vi "Update Measurement Details.vi"(8 "error in":errorcluster, 9 "measurement service description":string, 10 "measurement service name":string, 11 "project ref":refnum<vi>) -> (0 "error out":errorcluster, 3 "project ref out":refnum<vi>)   [LabVIEW 2021, in "MeasurementService Editor.lvlib"]
uses:
  MeasurementService Editor.lvlib
  Converter/Converter Reusables/Converter Reusables.lvlib
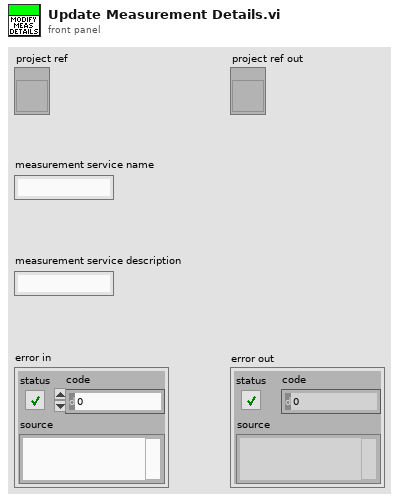
[diagram p1: front panel]
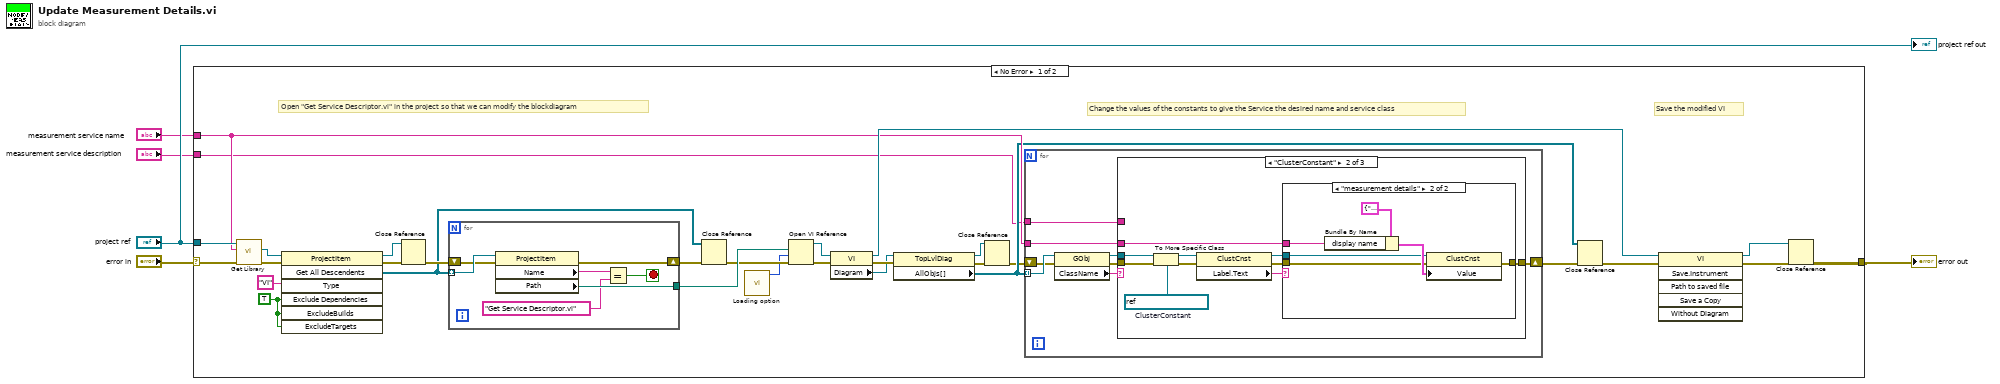
[diagram p0: block diagram]
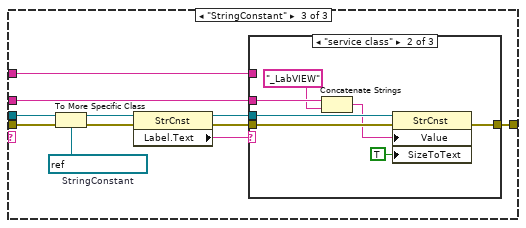
[diagram p4: hidden frame]
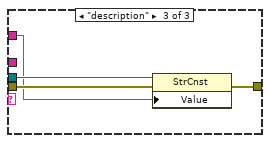
[diagram p6: hidden frame]
diagram:
  n1 = case shown="No Error" "error in" {
    selector: "error in" -> [w23 w92]
    tunnel: "project ref" -> [w22 _]
    tunnel: [w33 w92] -> w3
    tunnel: "measurement service name" -> [w16 _]
    tunnel: "measurement service description" -> [w9 _]
    frame No Error {
      w35 = TRUE ("ExcludeDependencies")
      # "Save the modified VI"
      # "Open \"Get Service Descriptor.vi\" in the project so that we can modify the blockdiagram"
      # "Change the values of the constants to give the Service the desired name and service class"
      n2 = call "Get Library.vi"("error in (no error)"=w23, "library name"=w16, "project ref"=w22) -> ("error out"=w21:errorcluster, "library item"=w20:refnum<vi>)  [unwired: 5 in, 2 out]
      n3 = invoke class="ProjectItem" method="Get All Descendents"(reference=w20, error in=w21, "Type"="VI", "Exclude Dependencies"=w35, "ExcludeBuilds"=w35, "ExcludeTargets"=w35) -> (reference out=w17:refnum<vi>, error out=w19:errorcluster, "All Descendents"=w7:refnum<vi>[])  [unwired: 1 in, 4 out]
      n4 = Close Reference(reference=w17, error in (no error)=w19) -> (error out=w18:errorcluster)
      n5 = for {
        tunnel: w7 -> [w91] mode=indexing
        shift-right: [w86] -> w14
        shift-left: w18 -> [w89]
        tunnel: [w87] -> w15
        stop <- w88 stop-if-true
        n6 = property class="ProjectItem"(reference=w91, error in=w89) -> (error out=w86:errorcluster, "Name"=w90:string, "Path"=w87:path)  [unwired: 1 out]
        n7 = Equal?(x=w90, y="Get Service Descriptor.vi") -> (x = y?=w88:bool)
      }
      n8 = Close Reference(reference=w7, error in (no error)=w14) -> (error out=w8:errorcluster)
      n9 = call "Loading option.vi"() -> ("options"=w6:i32)  [unwired: 11 in]
      n10 = Open VI Reference(vi path=w15, options=w6, error in (no error)=w8) -> (vi reference=w30:refnum<vi>, error out=w28:errorcluster)  [unwired: 3 in]
      n11 = property class="VI"(reference=w30, error in=w28) -> (reference out=w26:refnum<vi>, error out=w29:errorcluster, "Diagram"=w27:refnum<vi>)
      n12 = property class="TopLvlDiag"(reference=w27, error in=w29) -> (reference out=w10:refnum<vi>, error out=w12:errorcluster, "AllObjs[]"=w13:refnum<vi>[])
      n13 = Close Reference(reference=w10, error in (no error)=w12) -> (error out=w11:errorcluster)
      n14 = for {
        tunnel: w13 -> [w43] mode=indexing
        shift-right: [w37] -> w25
        shift-left: w11 -> [w42]
        tunnel: w16 -> [w38]
        tunnel: w9 -> [w36]
        n15 = property class="GObj"(reference=w43, error in=w42) -> (reference out=w40:refnum<vi>, error out=w39:errorcluster, "ClassName"=w41:string)
        n16 = case shown="\"ClusterConstant\"" w41 {
          tunnel: w40 -> [_ w53 w71]
          tunnel: w39 -> [w44 w52 w70]
          tunnel: w38 -> [_ w51 w63]
          tunnel: [w44 w50 w69] -> w37
          tunnel: w36 -> [_ _ w62]
          frame Default {
          }
          frame "ClusterConstant" {
            w54 = refnum<vi> refnum  # ClusterConstant
            n17 = To More Specific Class(target class=w54, reference=w53, error in=w52) -> (specific class reference=w49:refnum<vi>, error out=w48:errorcluster)
            n18 = property class="ClustCnst"(reference=w49, error in=w48) -> (reference out=w47:refnum<vi>, error out=w46:errorcluster, "Label.Text"=w45:string)
            n19 = case shown="\"measurement details\"" w45 {
              tunnel: w51 -> [_ w60]
              tunnel: [w55 w59] -> w50
              tunnel: w47 -> [_ w57]
              tunnel: w46 -> [w55 w56]
              frame Default {
              }
              frame "measurement details" {
                n20 = Bundle By Name(cluster=cluster{"display name":string, "version":string} {"display name"="Measurement Template", "version"="1.0.0"} ("ni_measurements_v1_MeasurementDetails"), "display name"=w60) -> (w58:cluster{"display name":string, "version":string})
                n21 = property class="ClustCnst"(reference=w57, error in=w56, "Value"=w58) -> (error out=w59:errorcluster)  [unwired: 1 out]
              }
            }
          }
          frame "StringConstant" {
            w72 = refnum<vi> refnum  # StringConstant
            n22 = To More Specific Class(target class=w72, reference=w71, error in=w70) -> (specific class reference=w68:refnum<vi>, error out=w67:errorcluster)
            n23 = property class="StrCnst"(reference=w68, error in=w67) -> (reference out=w65:refnum<vi>, error out=w64:errorcluster, "Label.Text"=w66:string)
            n24 = case shown="\"service class\"" w66 {
              tunnel: [w73 w80 w84] -> w69
              tunnel: w65 -> [_ w79 w83]
              tunnel: w64 -> [w73 w78 w82]
              tunnel: w63 -> [_ w77 _]
              tunnel: w62 -> [_ _ w81]
              frame Default {
              }
              frame "service class" {
                n25 = Concatenate Strings(w77, "_LabVIEW" ("string")) -> (w75:string)
                n26 = property class="StrCnst"(reference=w79, error in=w78, "Value"=w75, "SizeToText"=TRUE ("Size To Text?")) -> (error out=w80:errorcluster)  [unwired: 1 out]
              }
              frame "description" {
                n27 = property class="StrCnst"(reference=w83, error in=w82, "Value"=w81) -> (error out=w84:errorcluster)  [unwired: 1 out]
              }
            }
          }
        }
      }
      n28 = Close Reference(reference=w13, error in (no error)=w25) -> (error out=w24:errorcluster)
      n29 = invoke class="VI" method="Save.Instrument"(reference=w26, error in=w24) -> (reference out=w32:refnum<vi>, error out=w31:errorcluster)  [unwired: 4 in, 4 out]
      n30 = Close Reference(reference=w32, error in (no error)=w31) -> (error out=w33:errorcluster)
    }
    frame Error {
    }
  }
  "error out" <- w3
  "project ref out" <- "project ref"
